vi "Test Handle Error Passes Timeout.vi"(8 "error in (no error)":errorcluster) -> (0 "error out":errorcluster)   [LabVIEW 2019, in "RemoteControl.ZMQ.Tests.lvclass"]
uses:
  RemoteControl.ZMQ.Tests.lvclass
  <vilib>/addons/_JKI Toolkits/Caraya/classes/Assert/Assert.lvclass
  <vilib>/addons/_JKI Toolkits/Caraya/classes/Test/Test.lvclass
  src/RemoteControl.ZMQ/RemoteControl.ZMQ.lvclass
  <vilib>/addons/_JKI Toolkits/Caraya/classes/Assert/Assert True.vi
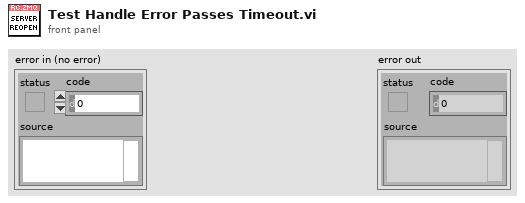
[diagram p1: front panel]
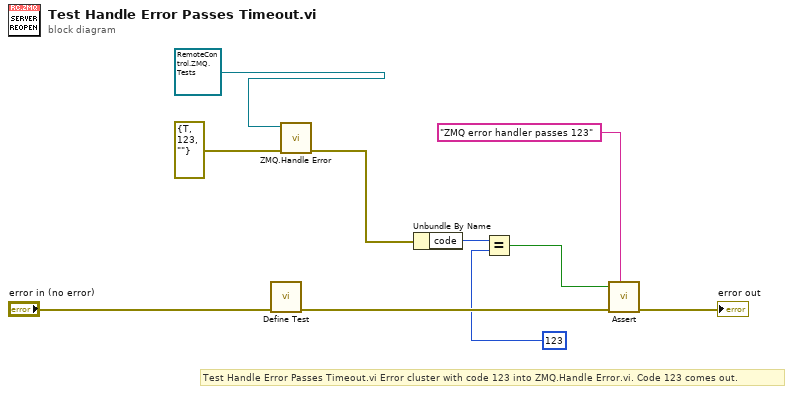
[diagram p0: block diagram]
diagram:
  # "Test Handle Error Passes Timeout.vi\tError cluster with code 123 into ZMQ.Handle Error.vi.\tCode 123 comes out."
  n1 = call <vilib>:"Define Test.vi"("error in (no error)"="error in (no error)") -> ("error out"=w7:errorcluster)  [unwired: 9 in, 1 out]
  n2 = call "ZMQ.Handle Error.vi"("error in (no error)"=errorcluster {"status"=TRUE, "code"=123, "source"=""}, "RemoteControl.ZMQ in"=refnum<class "RemoteControl.ZMQ.Tests.lvclass"> refnum ("RemoteControl.ZMQ.Tests.lvclass")) -> ("error out"=w3:errorcluster)  [unwired: 8 in, 1 out]
  n3 = Unbundle By Name(w3) -> ("code"=w5:i32)
  n4 = Equal?(x=w5, y=123 ("error code (1)")) -> (x = y?=w2:bool)
  n5 = call-poly <vilib>:"Assert.vi"("Label"="ZMQ error handler passes 123", "error in (no error)"=w7, "True?"=w2) -> ("error out"=→"error out":errorcluster)  [unwired: 7 in, 1 out]
